vi "Setting Database.Refresh.vi"(8 "error in (no error)":errorcluster, 10 "Initialize":T1, 11 "Setting Database":refnum<class "Setting Database.lvclass">) -> (0 "error out":errorcluster, 3 "Setting Database out":refnum<class "Setting Database.lvclass">)   [LabVIEW 2019, in "Setting Database.lvclass"]
doc: "This will reset the list of Objects. This will set it to how many you specify in the input. If there are existing settings at an index, it will use those settings. If there is no existing settings, then it will use the default settings, which are accessed from an INI file in the default Lithography location. This will trigger the Settings Database to publish the following information: The new lists of Path, Rectangle and Funnel settings, as well as the new active objects (Funnel, Path, Rectangle etc). The active object index will also be returned to zero, so make sure that you handle the necessary UI changes."
uses:
  Setting Database.lvclass
  Typedefs/PrivateEvents--Setting Database.Refresh.ctl
  Setting Database.lvclass/Setting Database.ctl
  Identity/Identifier.lvclass
  Tool/Tool Data/Tool Data/Tool Data.lvclass
panel:
  # "For instructions on how to use the JKI State Machine Objects, examples and video tutorials, visit:\nhttp://jki.net/state-machine-objects/\n\nJKI State Machine Objects™\nhttp://jki.net/state-machine-objects/\nCopyright (C) 2005-2015, JKI <info@jki.net>\nALL RIGHTS RESERVED"
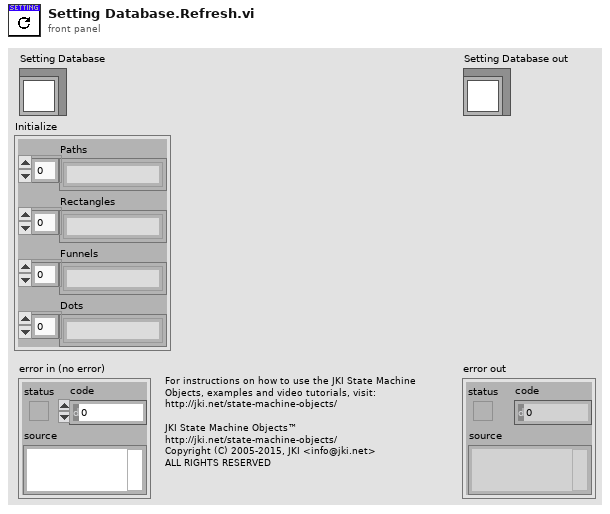
[diagram p1: front panel]
types:
  T1 = typedef "Setting Database.lvclass/PrivateEvents--Setting Database.Refresh.ctl" = cluster{"Paths":string[], "Rectangles":string[], "Funnels":string[], "Dots":string[]}
  T2 = cluster{"paths":string[], "funnels":string[], "rects":string[], "dots":string[]}
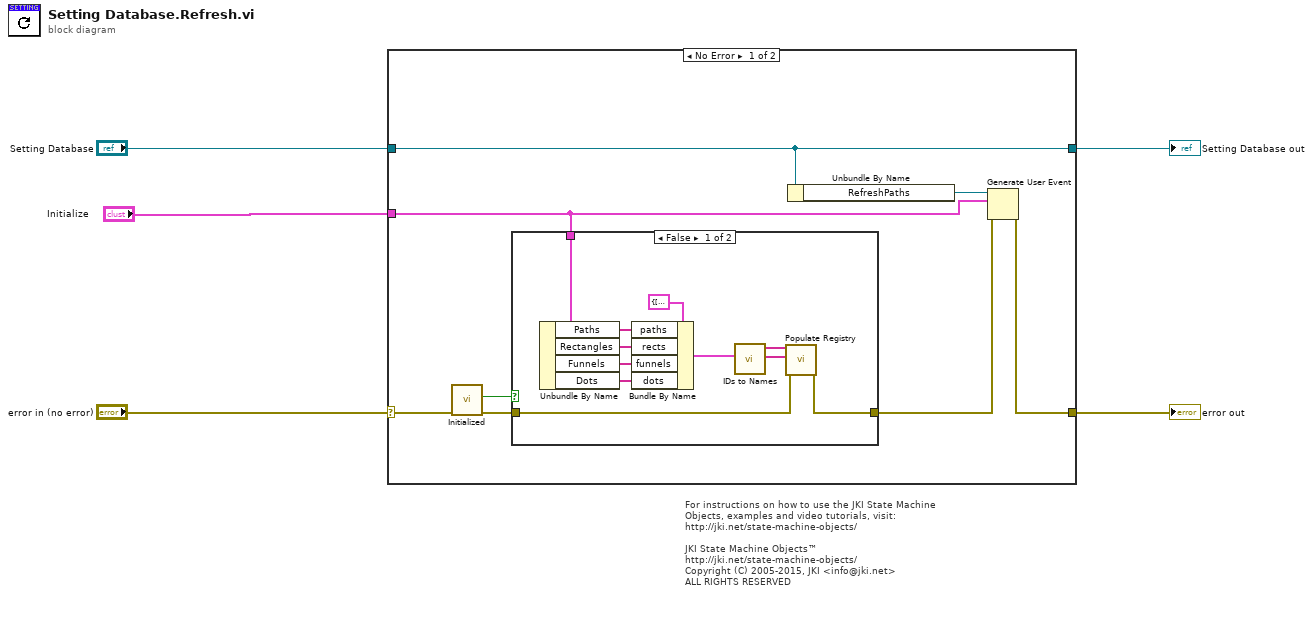
[diagram p0: block diagram]
diagram:
  # "For instructions on how to use the JKI State Machine Objects, examples and video tutorials, visit:\nhttp://jki.net/state-machine-objects/\n\nJKI State Machine Objects™\nhttp://jki.net/state-machine-objects/\nCopyright (C) 2005-2015, JKI <info@jki.net>\nALL RIGHTS RESERVED"
  n1 = case shown="No Error" "error in (no error)" {
    selector: "error in (no error)" -> [w10 w27]
    tunnel: [w12 w27] -> w4
    tunnel: [w11 w26] -> w5
    tunnel: "Setting Database" -> [w11 w26]
    tunnel: "Initialize" -> [w9 _]
    frame No Error {
      n2 = call "Initialized.vi"("error in"=w10) -> ("error out"=w8:errorcluster, "Initialized?"=w6:bool)  [unwired: 9 in]
      n3 = case shown="False" w6 {
        tunnel: w9 -> [w24 _]
        tunnel: w8 -> [w15 w25]
        tunnel: [w14 w25] -> w7
        frame False {
          n4 = Unbundle By Name(w24) -> ("Paths"=w21:string[], "Rectangles"=w20:string[], "Funnels"=w19:string[], "Dots"=w18:string[])
          n5 = Bundle By Name(cluster=T2 {"paths"=[], "funnels"=[], "rects"=[], "dots"=[]} ("IDs"), "paths"=w21, "rects"=w20, "funnels"=w19, "dots"=w18) -> (w22:T2)
          n6 = call "IDs to Names.vi"("IDs"=w22) -> ("Names"=w16:string[], "IDs"=w17:string[])  [unwired: 9 in]
          n7 = call "Populate Registry.vi"("error in"=w15, "Aliases"=w16, "Names"=w17) -> ("error out"=w14:errorcluster)  [unwired: 8 in]
        }
        frame True {
        }
      }
      n8 = Unbundle By Name(w11) -> ("RefreshPaths"=w13:refnum<user-event>)
      n9 = Generate User Event(user event=w13, event data cluster=w9, error in=w7) -> (error out=w12:errorcluster)  [unwired: 1 in, 1 out]
    }
    frame Error {
    }
  }
  "error out" <- w4
  "Setting Database out" <- w5
